vi "Clear Trace.vi"(8 "error in (no error)":errorcluster caption="에러 입력(에러 없음)", 11 "Instrument Manager 입력":refnum<class "Instrument Manager.lvclass">) -> (0 "error out":errorcluster caption="에러 출력", 3 "Instrument Manager 출력":refnum<class "Instrument Manager.lvclass">)   [LabVIEW 2023, in "Instrument Manager.lvclass"]
uses:
  Instrument Manager.lvclass
  Instrument Manager.lvclass/Instrument Manager.ctl
  Module/Spectrum Analyzer/TYPE DEFINITION/TYPE Display Trace Mode Select.ctl
  Module/Spectrum Analyzer/Spectrum Analyzer.lvlib
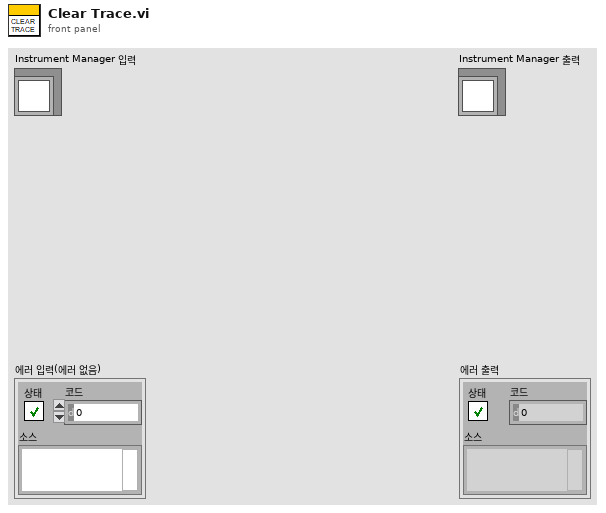
[diagram p1: front panel]
types:
  T1 = typedef "Spectrum Analyzer.lvlib/TYPE Display Trace Mode Select.ctl" = enum16{"Clear Write", "Max Hold", "Min Hold", "Average", "View"}
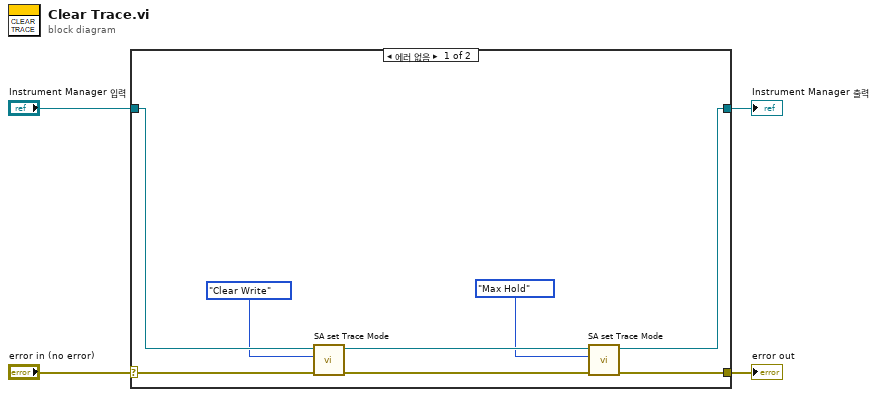
[diagram p0: block diagram]
diagram:
  n1 = case shown="에러 없음" "error in (no error)" {
    selector: "error in (no error)" -> [w12 w14]
    tunnel: [w10 w14] -> w3
    tunnel: [w6 w13] -> w1
    tunnel: "Instrument Manager 입력" -> [w9 w13]
    frame No Error {
      n2 = call "SA set Trace Mode.vi"("error in (no error)"=w12, "Trace Mode"=TYPE_Display_Trace_Mode_Select."Clear Write", "Instrument Manager 입력"=w9) -> ("error out"=w11:errorcluster, "Instrument Manager 출력"=w7:refnum<class "Instrument Manager.lvclass">)  [unwired: 7 in]
      n3 = call "SA set Trace Mode.vi"("error in (no error)"=w11, "Trace Mode"=TYPE_Display_Trace_Mode_Select."Max Hold", "Instrument Manager 입력"=w7) -> ("error out"=w10:errorcluster, "Instrument Manager 출력"=w6:refnum<class "Instrument Manager.lvclass">)  [unwired: 7 in]
    }
    frame Error {
    }
  }
  "error out" <- w3
  "Instrument Manager 출력" <- w1
